vi "FuncVI_Sub - WFGraph - Master.vi"() -> ()   [LabVIEW 2021]
doc: "::: CalcExpress Toolkit :::\nCopyright (c) 2000-2026 Konstantin Shifershteyn. All rights reserved."
panel:
  in  "data":string
  in  "update":bool
  out "graph":cluster{dbl, dbl, "Sine Wave":dbl[]}[](graph)
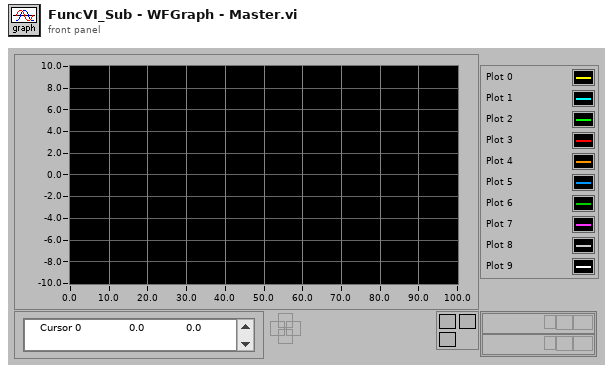
[diagram p1: front panel]
types:
  T1 = typedef "LVRectTypeDef.ctl" = cluster{"Left":i16, "Top":i16, "Right":i16, "Bottom":i16}
  T2 = cluster{"plot":i32, "Y":dbl[], "x0":dbl, "dx":dbl, "plot name":string}
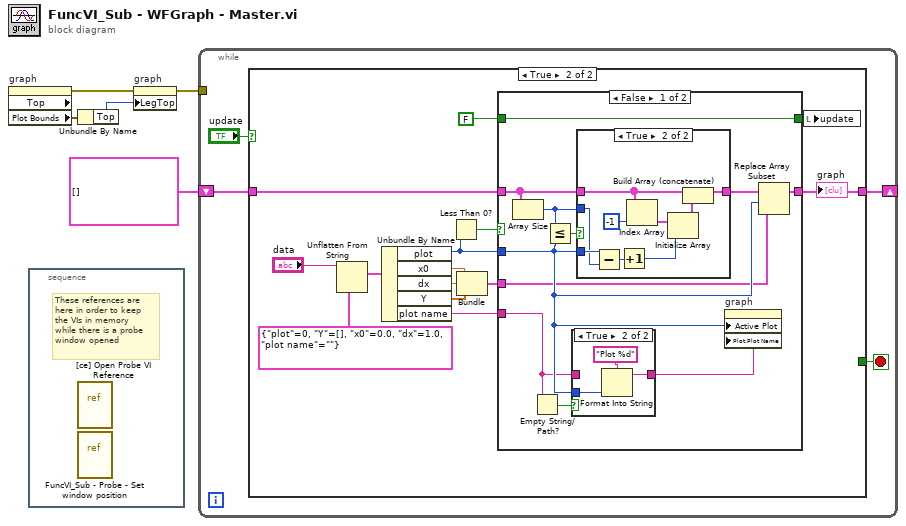
[diagram p0: block diagram]
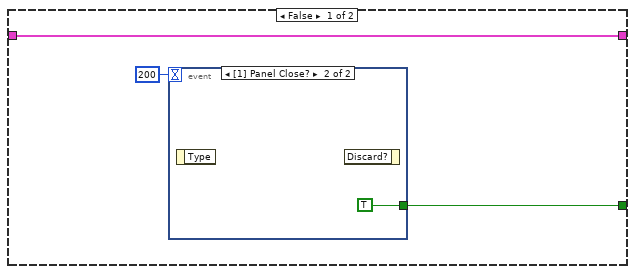
[diagram p2: hidden frame]
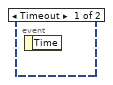
[diagram p3: hidden frame]
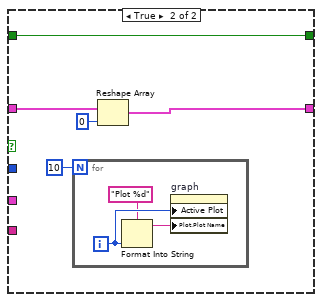
[diagram p6: hidden frame]
diagram:
  n1 = property on="graph" class="WFGraph (strict)" props=["Top", "Plot Bounds"]() -> (error out=w4:errorcluster, "Plot Bounds"=w2:T1)  [unwired: 2 in, 2 out]
  n2 = stacked-sequence {
    frame #0 {
      # "These references are\nhere in order to keep\nthe VIs in memory\nwhile there is a probe\nwindow opened"
      n3 = vi-ref "[ce] Open Probe VI Reference.vi"() -> ()  [unwired: 1 out]
      n4 = vi-ref "FuncVI_Sub - Probe - Set window position.vi"() -> ()  [unwired: 1 out]
    }
  }
  n5 = Unbundle By Name(w2) -> ("Top"=w1:i16)
  n6 = property on="graph" class="WFGraph (strict)"(error in=w4, "LegTop"=w1) -> (error out=w3:errorcluster)  [unwired: 1 in, 1 out]
  n7 = while {
    shift-right: [w8] -> _
    shift-left: cluster{dbl, dbl, "Sine Wave":dbl[]}[] [] -> [w7]
    tunnel: w3 -> [_]
    stop <- w6 stop-if-true
    n8 = case shown="True" "update" {
      tunnel: [w12 w17] -> w8
      tunnel: w7 -> [w12 w16]
      tunnel: [w10 _] -> w6
      frame False {
        n9 = event shown="[1] Panel Close?" {
          selector: _ -> [_ _]
          dyn-events: _ -> [_ _]
          timeout: 200 -> [_ _]
          tunnel: [_ TRUE] -> w10
          event Timeout {
            n10 = event-data() -> ()  [unwired: 1 in, 1 out]
          }
          event Panel Close? {
            n11 = event-data() -> ()  [unwired: 1 in, 1 out]
            n12 = event-data() -> ()  [unwired: 2 in, 1 out]
          }
        }
      }
      frame True {
        n13 = Unflatten From String(type=T2 {"plot"=0, "Y"=[], "x0"=0.0, "dx"=1.0, "plot name"=""}, binary string="data") -> (value=w24:T2)  [unwired: 3 in, 2 out]
        n14 = Unbundle By Name(w24) -> ("plot"=w19:i32, "x0"=w23:dbl, "dx"=w22:dbl, "Y"=w21:dbl[], "plot name"=w20:string)
        n15 = Less Than 0?(x=w19) -> (x < 0?=w27:bool)
        n16 = Bundle("x0"=w23, "dx"=w22, "Y"=w21) -> (w18:cluster{"x0":dbl, "dx":dbl, "Y":dbl[]})  [unwired: 1 in]
        n17 = case shown="False" w27 {
          tunnel: w19 -> [w34 _]
          tunnel: [w35 w53] -> w17
          tunnel: w20 -> [w31 _]
          tunnel: w18 -> [w30 _]
          tunnel: w16 -> [w29 w55]
          tunnel: FALSE ("update") -> [w28 w56]
          tunnel: [w28 w56] -> w15
          frame False {
            n18 = Array Size(array=w29) -> (size(s)=w37:i32)
            n19 = Empty String/Path?(string/path=w31) -> (empty?=w32:bool)
            n20 = Less Or Equal?(x=w37, y=w34) -> (x <= y?=w38:bool)
            n21 = case shown="True" w32 {
              tunnel: w34 -> [_ w41]
              tunnel: [w39 w40] -> w33
              tunnel: w31 -> [w39 _]
              frame False {
              }
              frame True {
                n22 = Format Into String(format string="Plot %d", w41) -> (resulting string=w40:string)  [unwired: 2 in, 1 out]
              }
            }
            n23 = case shown="True" w38 {
              tunnel: w29 -> [w43 w45]
              tunnel: w34 -> [_ w52]
              tunnel: [w43 w47] -> w36
              tunnel: w37 -> [_ w51]
              frame False {
              }
              frame True {
                n24 = Subtract(x=w52, y=w51) -> (x-y=w50:i32)
                n25 = Increment(x=w50) -> (x+1=w49:i32)
                n26 = Index Array(array=w45, index=-1) -> (element=w46:cluster{dbl, dbl, "Sine Wave":dbl[]})
                n27 = Initialize Array(w46, w49) -> (w48:cluster{dbl, dbl, "Sine Wave":dbl[]}[])
                n28 = Build Array (concatenate)(w45, w48) -> (w47:cluster{dbl, dbl, "Sine Wave":dbl[]}[])
              }
            }
            n29 = property on="graph" class="WFGraph (strict)"("Active Plot"=w34, "Plot.Plot Name"=w33) -> ()  [unwired: 2 in, 2 out]
            n30 = Replace Array Subset(array=w36, new element=w30, index=w34) -> (w35:cluster{dbl, dbl, "Sine Wave":dbl[]}[])
          }
          frame True {
            n31 = for {
              N: 10 -> [_]
              i -> [w59]
              n32 = Format Into String(format string="Plot %d", w59) -> (resulting string=w60:string)  [unwired: 2 in, 1 out]
              n33 = property on="graph" class="WFGraph (strict)"("Active Plot"=w59, "Plot.Plot Name"=w60) -> ()  [unwired: 2 in, 2 out]
            }
            n34 = Reshape Array(w55, 0 ("dimension size")) -> (w53:cluster{dbl, dbl, "Sine Wave":dbl[]}[])
          }
        }
        "graph" <- w17
        n35 = local write "update"(w15) -> ()
      }
    }
  }
